vi "ClassAttributes_AddClassAttributes.vi"(7 "Action":T3=enum."GeneratePattern", 8 "error in (no error)":errorcluster, 10 "DataIn":variant, 11 "ClassRefToActOn":refnum<vi>) -> (0 "error out":errorcluster, 1 "Name":string, 2 "DataOut":variant, 3 "Cancelled":bool)   [LabVIEW 2020]
uses:
  Provider_BaseClassInterface/BaseProvider_SubVIs/BaseProvider_DesignPatternsActions.ctl
  Common/CommonVIs/CommonVIs_AttributeDataType.ctl
  Common/LvClass_class/GDSLvClass_ProviderTypes.ctl
  Provider_EndevoGOOP400/EndevoG4ProviderName.ctl
  Common/ScriptingFunctions/Scripting_ConnectorPanePatternType.ctl
  <vilib>/picture/picture.llb/imagedata.ctl
  Provider_LvNativeClass/ClassWriterNative_class/ClassWriterNative.lvclass
  Provider_BaseClassInterface/CreateMethodData.ctl
  Provider_EndevoGOOP300/GOOP300_SubVIs/GOOP300_MethodScopeType.ctl
  Provider_LvNativeClass/ClassWriterNative_class/IconDetails.ctl
  Provider_LvNativeClass/ClassWriterNative_class/IconSize.ctl
  Provider_BaseClassInterface/ClassWriter_class/ClassWriter.lvclass
panel:
  in  "_Cancel":bool
  in  "_OK":bool
  in  "ProcessName":T2(array[cluster]) caption="Attributes to add (can be empty)\nName                                        Array?      Data Type" {"Array?" items=["No", "1D", "2D", "3D"]}
  # "Class Attributes"
  # "Create"
  # "Get"
  # "Set"
  # "method"
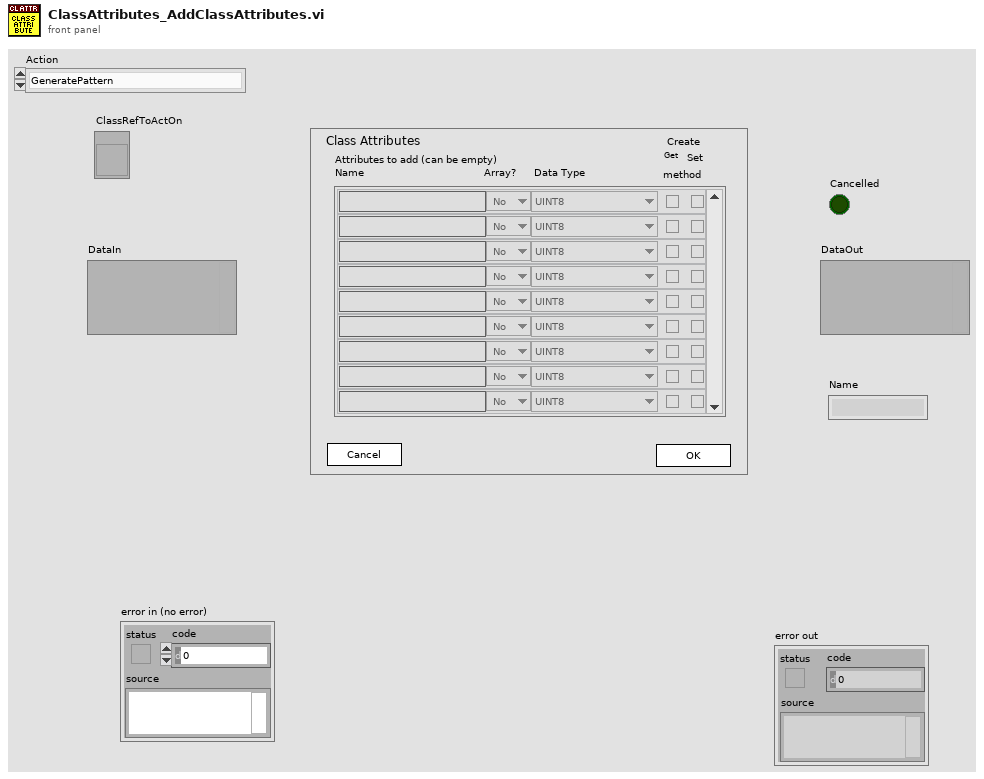
[diagram p1: front panel]
types:
  T1 = typedef "CommonVIs_AttributeDataType.ctl" = enum16{"UINT8", "INT8", "UINT16", "INT16", "UINT32", "INT32", "UINT64", "INT64", "SGL", "DBL", "EXT", "CSG", "CDB", "CXT", "TimeStamp", "STRING", "PATH", "BOOL", "ENUM", "RefNum", "VIRefNum", "LabVIEW Class", "Cluster", "Variant", "TypeDef", "Waveform", "LabVIEW Object", "Other", "void", "Set", "Map"}
  T2 = cluster{"Name":string, "Array?":u16, "AttributeDataType":T1, "GetMethod":bool, "SetMethod":bool}[]
  T3 = typedef "BaseProvider_DesignPatternsActions.ctl" = enum16{"AddPatternDialog", "GeneratePattern", "RemovePattern", "CreatePatternMethod", "UpdatePattern"}
  T4 = typedef "GDSLvClass_ProviderTypes.ctl" = enum16{"UnKnown(LabVOOP)", "Native", "EndevoGOOP3", "OpenG(RootObject)", "OpenG(OpenG_Object)", "EndevoGOOP4", "JKI1"}
  T5 = cluster{"Application":refnum<vi>, "SupportFolder":path, "TemplateName":string, "ClassProvider":T4, "ProtectedFolder":path, "UtilsFolder":path, "ProtectedFolderRef":refnum<vi>, "UtilsFolderRef":refnum<vi>, "ClassName":string, "GetClassAttributes.vi":path, "ClassAttributes.ctl":path, "GetClassAttributesRef":refnum<vi>, "ClassAttributesRef":refnum<vi>, "ProcessIdRef":refnum<vi>, "Data":cluster{"Name":string, "Array?":u16, "AttributeDataType":T1, "GetMethod":bool, "SetMethod":bool}[], "Singleton":bool, "VI_ToFind":path, "MethodTemplate":path, "VI":refnum<vi>, "GetObjectStatus":path, "ClassAttrib":refnum<vi>}
  T6 = cluster{"ProcessName":cluster{"Name":string, "Array?":u16, "AttributeDataType":T1, "GetMethod":bool, "SetMethod":bool}[]}
  T7 = cluster{"Cancelled":bool, "Files":path[], "ClassPath":path, "DataOut":variant}
  T8 = typedef "EndevoG4ProviderName.ctl" = enum16{"EndevoGOOP400"}
  T9 = enum32{"invalid lock state", "Not Locked", "Locked (No Password)", "Password-protected"}
  T10 = typedef "imagedata.ctl" = cluster{"image type":i32, "image depth":i32, "image":u8[], "mask":u8[], "colors":u32[], "Rectangle":cluster{"left":i16, "top":i16, "right":i16, "bottom":i16}}
  T11 = cluster{"AttributeNames":string[], "PropertyNode":bool, "FolderNames":string[]}
  T12 = typedef "ClassWriter.lvclass/CreateMethodData.ctl" = cluster{"MethodName":string, "RelativeMethodPath":path, "MethodDescription":string, "Scope/Visibility":T13, "MethodTemplateName":string, "IconOut":u8[][], "RelativeProjectClassPath":string, "OpenViAfterCreation":bool, "DynamicDispatchVi":bool, "ExtraCreateParameters":variant, "MustOverride":bool, "MustCallParent":bool, "IconDetails":T14, "AF-Option":variant, "TemplatePath":path}
  T13 = typedef "GOOP300_MethodScopeType.ctl" = enum16{"Use Parent Folder Scope", "Public", "Protected", "Private", "Community"}
  T14 = typedef "ClassWriterNative.lvclass/IconDetails.ctl" = cluster{"IconSize":T15, "ImageRows(32)":i32, "ConnectorPaneHeight":i32[]}
  T15 = typedef "ClassWriterNative.lvclass/IconSize.ctl" = enum16{"Full", "1 c-term high", "2 c-term high", "3 c-term high"}
  T16 = typedef "GDSLvCLass_ClassSettingsType.ctl" = cluster{"ClassProviderName":string, "ClassTemplateUsed":string, "ClassTemplateVersion":string, "ClassDescription":string, "PlugIns":T17[], "ConnectorPanePattern":string}
  T17 = typedef "GDSLvClass_PlugIn.ctl" = cluster{"Type":T18, "ID":string, "Version":string, "Path":path, "Name":string, "Data":variant}
  T18 = typedef "GDSLvClass_PlugInTypes.ctl" = enum16{"DesignPattern", "MethodTypes"}
  T19 = enum32{"invalid scope", "public", "private", "protected"}[]
  T20 = typedef "GOOP400_Options.ctl" = cluster{"FlatFolderStructure":bool}
  T21 = typedef "Scripting_ConnectorPanePatternType.ctl" = u16
  T22 = typedef "GDSLvClass_IconSettingsType.ctl" = cluster{"Frame":u32, "Frame thickness":u8, "Header Background":u32, "Header Text":u32, "ColorPublic":u32, "ColorProtected":u32, "ColorPrivate":u32, "Body Text":u32, "ClassBodyIcon":string}
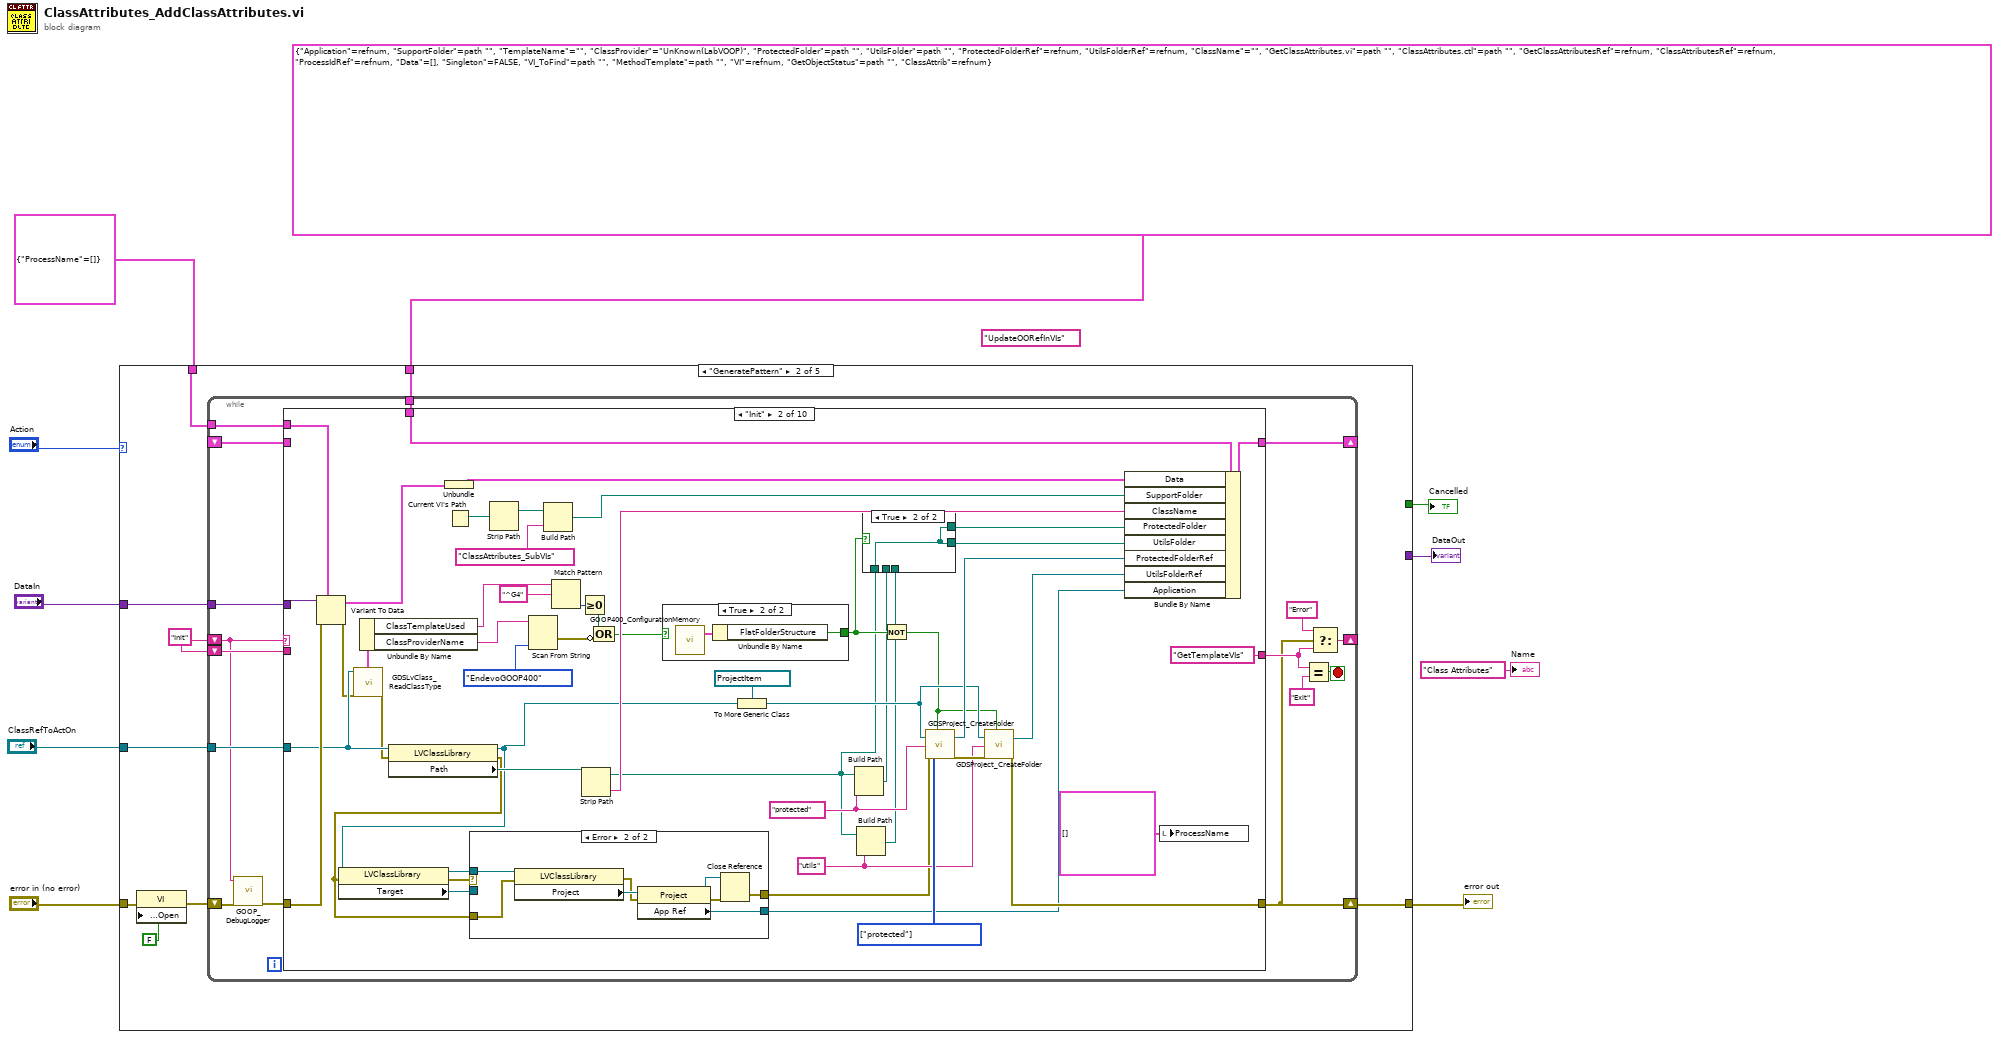
[diagram p0: block diagram]
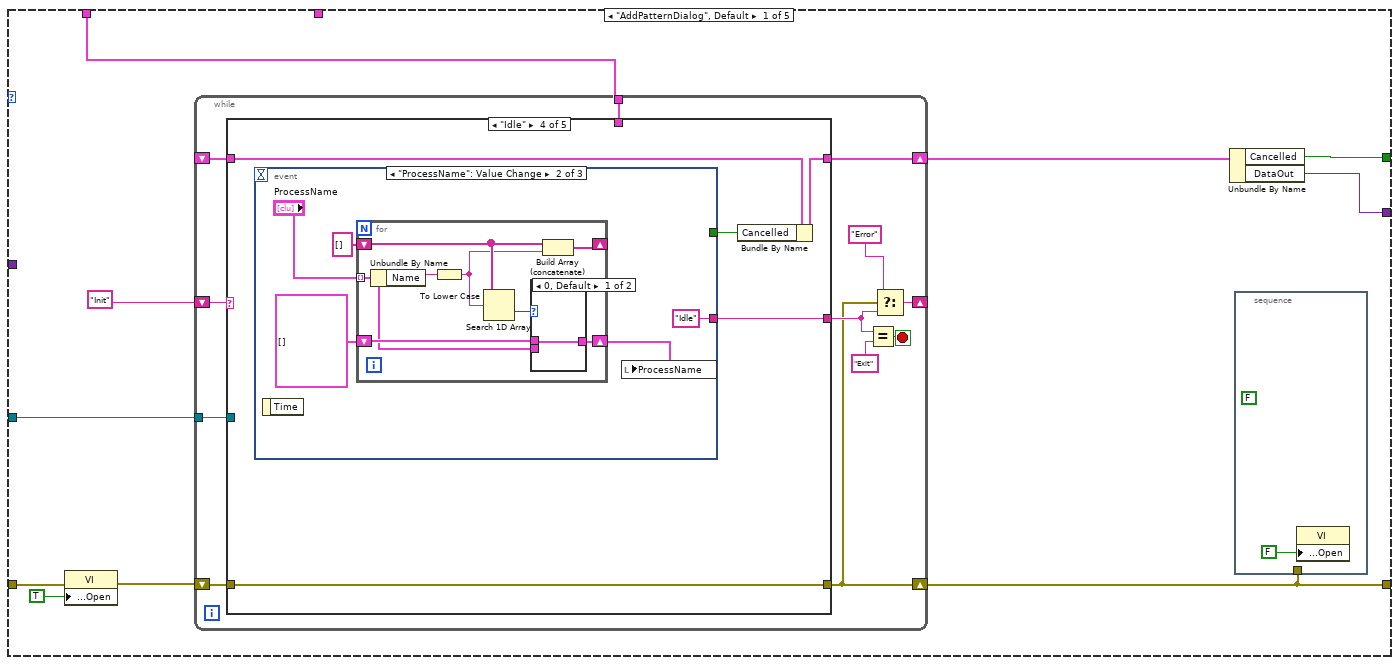
[diagram p2: hidden frame]
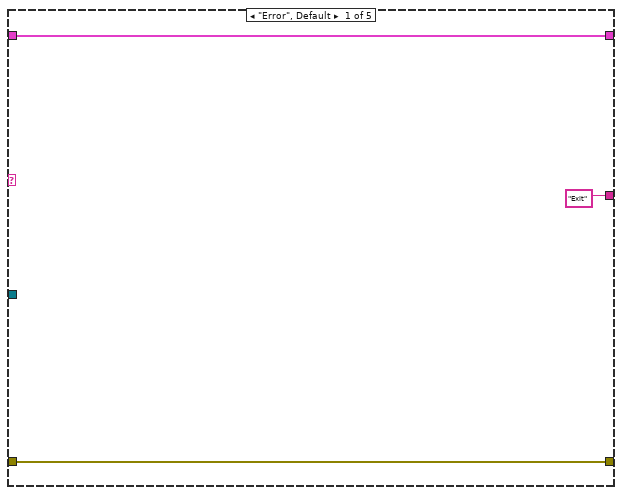
[diagram p3: hidden frame]
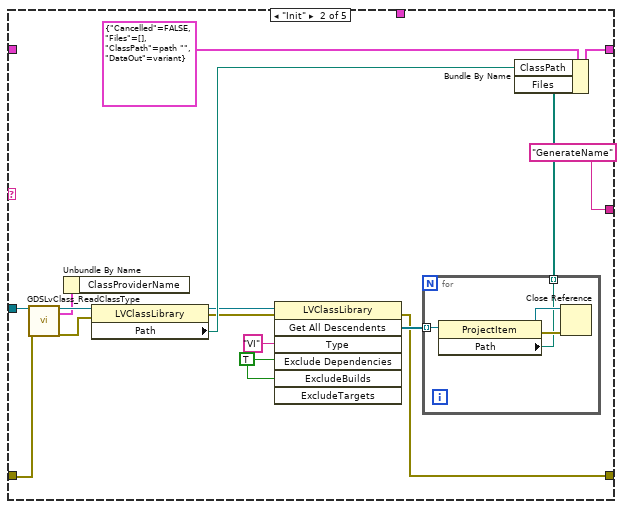
[diagram p4: hidden frame]
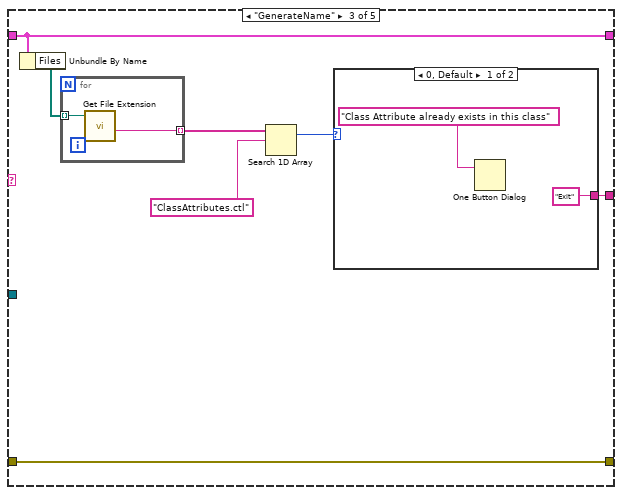
[diagram p5: hidden frame]
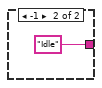
[diagram p6: hidden frame]
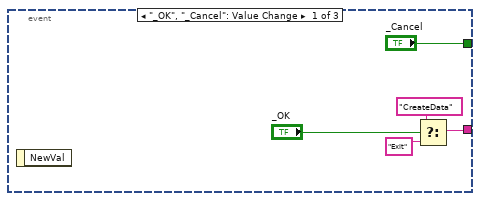
[diagram p7: hidden frame]
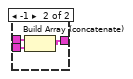
[diagram p8: hidden frame]
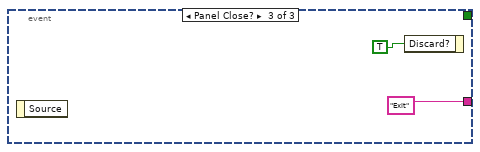
[diagram p9: hidden frame]
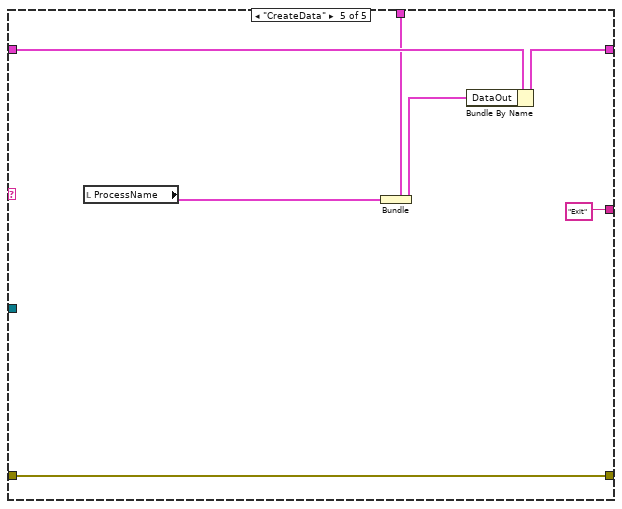
[diagram p10: hidden frame]
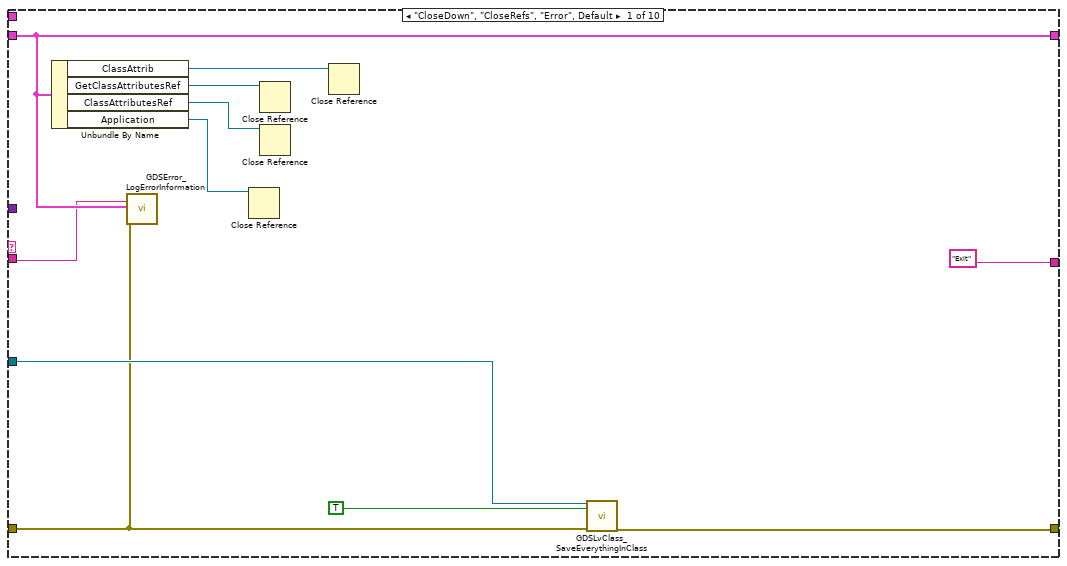
[diagram p11: hidden frame]
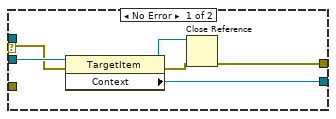
[diagram p14: hidden frame]
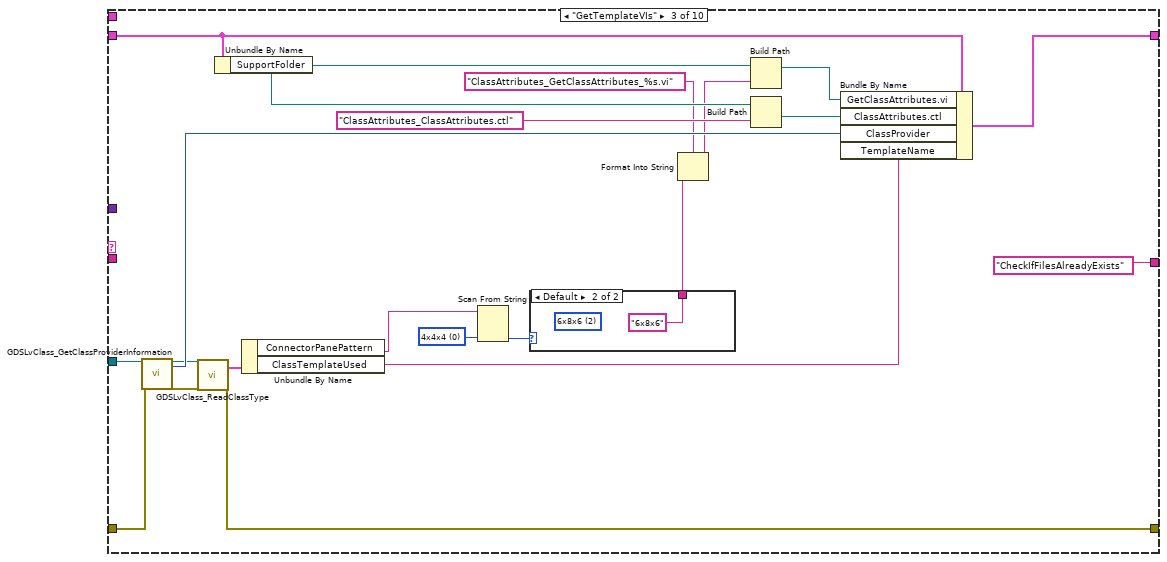
[diagram p15: hidden frame]
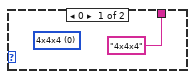
[diagram p16: hidden frame]
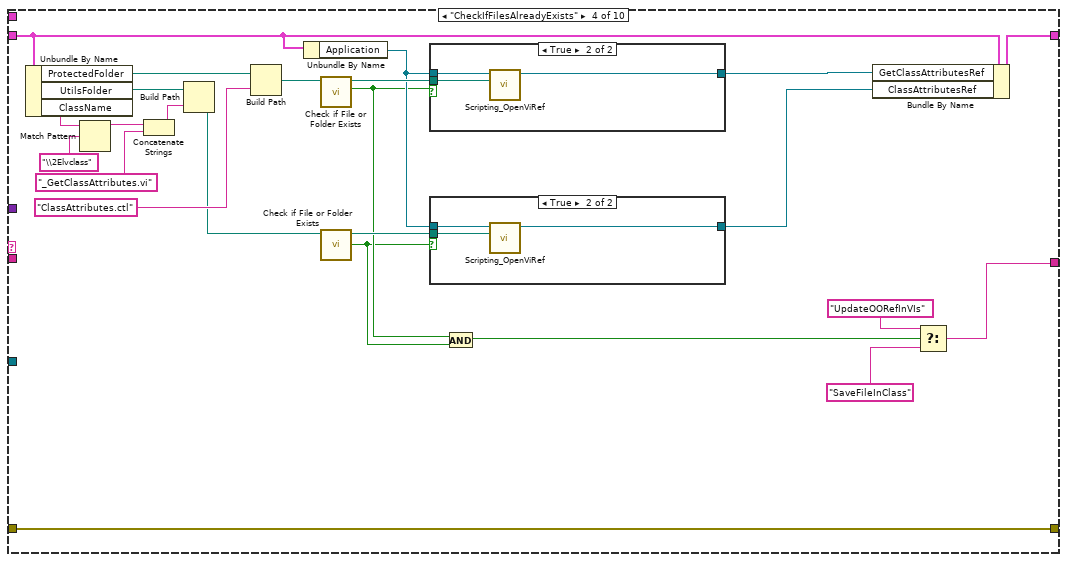
[diagram p17: hidden frame]
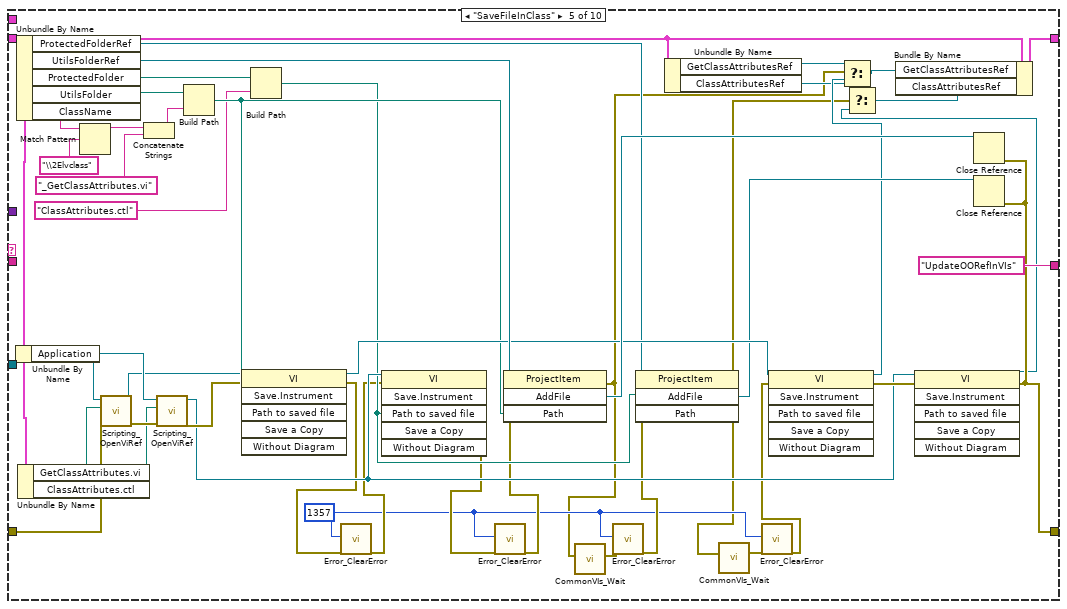
[diagram p20: hidden frame]
diagram:
  (unwired) "UpdateOORefInVIs"
  n1 = case shown="\"GeneratePattern\"" "Action" {
    tunnel: "error in (no error)" -> [w19 w107 w556 w647 w648]
    tunnel: [w16 w113 w562 w647 w648] -> w8
    tunnel: "ClassRefToActOn" -> [w14 w109 w558 _ _]
    tunnel: [w13 _ _ _ _] -> w6
    tunnel: [w12 _ _ _ _] -> w5
    tunnel: T6 {"ProcessName"=[]} ("output cluster") -> [w11 w111 w560 _ _]
    tunnel: "DataIn" -> [_ w112 w561 _ _]
    tunnel: T5 {"Application"=refnum, "SupportFolder"=path "", "TemplateName"="", "ClassProvider"=enum."UnKnown(LabVOOP)", "ProtectedFolder"=path "", "UtilsFolder"=path "", "ProtectedFolderRef"=refnum, "UtilsFolderRef"=refnum, "ClassName"="", "GetClassAttributes.vi"=path "", "ClassAttributes.ctl"=path "", "GetClassAttributesRef"=refnum, "ClassAttributesRef"=refnum, "ProcessIdRef"=refnum, "Data"=[], "Singleton"=FALSE, "VI_ToFind"=path "", "MethodTemplate"=path "", "VI"=refnum, "GetObjectStatus"=path "", "ClassAttrib"=refnum} -> [_ w110 w559 _ _]
    frame "AddPatternDialog", Default {
      n2 = property class="VI"(error in=w19, "Front Panel.Open"=TRUE ("Front Panel Window:Open")) -> (error out=w18:errorcluster)  [unwired: 1 in, 1 out]
      n3 = while {
        shift-right: [w26] -> w16
        shift-left: w18 -> [w33]
        shift-right: [w31] -> _
        shift-left: "Init" -> [w32]
        shift-right: [w25] -> w15
        shift-left: _ -> [w24]
        tunnel: w14 -> [w23]
        tunnel: w11 -> [w22]
        stop <- w30 stop-if-true
        n4 = case shown="\"Idle\"" w32 {
          tunnel: w33 -> [w36 w39 w60 w72 w100]
          tunnel: [w36 w48 w60 w72 w100] -> w26
          tunnel: ["Exit" "GenerateName" w62 w73 "Exit"] -> w27
          tunnel: [w34 w46 w61 w71 w102] -> w25
          tunnel: w24 -> [w34 _ w61 w69 w104]
          tunnel: w23 -> [_ w41 _ _ _]
          tunnel: w22 -> [_ _ _ _ w99]
          frame "Error", Default {
          }
          frame "Init" {
            w50 = TRUE ("ExcludeDependencies")
            n5 = call "GDSLvClass_ReadClassType.vi"("Class Refnum In"=w41, "error in (no error)"=w39) -> ("Class Refnum Out"=w40:refnum<vi>, "ClassSettings"=w37:T16, "error out"=w38:errorcluster)  [unwired: 15 in]
            n6 = Unbundle By Name(w37) -> ()  [unwired: 1 out]
            n7 = property class="LVClassLibrary"(reference=w40, error in=w38) -> (reference out=w43:refnum<vi>, error out=w42:errorcluster, "Path"=w45:path)
            n8 = invoke class="LVClassLibrary" method="Get All Descendents"(reference=w43, error in=w42, "Type"="VI", "Exclude Dependencies"=w50, "ExcludeBuilds"=w50) -> (error out=w48:errorcluster, "All Descendents"=w49:refnum<vi>[])  [unwired: 2 in, 5 out]
            n9 = for {
              tunnel: w49 -> [w56] mode=indexing
              tunnel: [w53] -> w44 mode=indexing
              n10 = property class="ProjectItem"(reference=w56) -> (reference out=w54:refnum<vi>, error out=w55:errorcluster, "Path"=w53:path)  [unwired: 1 in]
              n11 = Close Reference(reference=w54, error in (no error)=w55) -> ()  [unwired: 1 out]
            }
            n12 = Bundle By Name(cluster=T7 {"Cancelled"=FALSE, "Files"=[], "ClassPath"=path "", "DataOut"=variant}, "ClassPath"=w45, "Files"=w44) -> (w46:T7)
          }
          frame "GenerateName" {
            n13 = Unbundle By Name(w61) -> ("Files"=w63:path[])
            n14 = for {
              tunnel: w63 -> [w68] mode=indexing
              tunnel: [w67] -> w59 mode=indexing
              n15 = call <vilib>:"Get File Extension.vi"("file"=w68) -> ("filename without extension"=w67:string)  [unwired: 6 in, 4 out]
            }
            n16 = Search 1D Array(1D array=w59, element="ClassAttributes.ctl") -> (index of element=w57:i32)  [unwired: 1 in]
            n17 = case shown="0, Default" w57 {
              tunnel: ["Exit" "Idle"] -> w62
              frame 0, Default {
                n18 = One Button Dialog(message="Class Attribute already exists in this class") -> ()  [unwired: 1 in, 1 out]
              }
              frame -1 {
              }
            }
          }
          frame "Idle" {
            n19 = event shown="[1] \"ProcessName\": Value Change" {
              selector: _ -> [_ _ _]
              dyn-events: _ -> [_ _ _]
              timeout: _ -> [_ _ _]
              tunnel: [w77 "Idle" "Exit"] -> w73
              tunnel: ["_Cancel" _ _] -> w70
              event "_OK", "_Cancel": Value Change {
                n20 = event-data() -> ()  [unwired: 1 in, 1 out]
                n21 = Select(t="CreateData", s="_OK", f="Exit") -> (s? t:f=w77:string)
              }
              event "ProcessName": Value Change {
                n22 = event-data() -> ()  [unwired: 1 in, 1 out]
                n23 = for {
                  tunnel: "ProcessName" -> [w85] mode=indexing
                  shift-right: [w91] -> _
                  shift-left: string[] [] -> [w89]
                  shift-right: [w84] -> w79
                  shift-left: T2 [] -> [w86]
                  n24 = Unbundle By Name(w85) -> ("Name"=w90:string)
                  n25 = To Lower Case(string=w90) -> (all lower case string=w88:string)
                  n26 = Search 1D Array(1D array=w89, element=w88) -> (index of element=w87:i32)  [unwired: 1 in]
                  n27 = case shown="0, Default" w87 {
                    tunnel: w86 -> [w92 w95]
                    tunnel: w85 -> [_ w94]
                    tunnel: [w92 w93] -> w84
                    frame 0, Default {
                    }
                    frame -1 {
                      n28 = Build Array (concatenate)(w95, w94) -> (w93:T2)
                    }
                  }
                  n29 = Build Array (concatenate)(w89, w88) -> (w91:string[])
                }
                n30 = local write "ProcessName"(w79) -> ()
              }
              event Panel Close? {
                n31 = event-data() -> ()  [unwired: 1 in, 1 out]
                n32 = event-data("Discard?"=TRUE) -> ()  [unwired: 1 in, 1 out]
              }
            }
            n33 = Bundle By Name(cluster=w69, "Cancelled"=w70) -> (w71:T7)
          }
          frame "CreateData" {
            n34 = local read "ProcessName"() -> (w98:T2)
            n35 = Bundle(cluster=w99, "ProcessName"=w98) -> (w103:T6)
            n36 = Bundle By Name(cluster=w104, "DataOut"=w103) -> (w102:T7)
          }
        }
        n37 = Equal?(x=w27, y="Exit") -> (x = y?=w30:bool)
        n38 = Select(t="Error", s=w26, f=w27) -> (s? t:f=w31:string)
      }
      n39 = Unbundle By Name(w15) -> ("Cancelled"=w13:bool, "DataOut"=w12:variant)
      n40 = stacked-sequence {
        tunnel: w16 -> [_]
        frame #0 {
          (unwired) FALSE ("Visible")
          n41 = property class="VI"("Front Panel.Open"=FALSE ("Front Panel Window:Open")) -> ()  [unwired: 2 in, 2 out]
        }
      }
    }
    frame "GeneratePattern" {
      w105 = "Init"
      n42 = property class="VI"(error in=w107, "Front Panel.Open"=FALSE ("Front Panel Window:Open")) -> (error out=w106:errorcluster)  [unwired: 1 in, 1 out]
      n43 = while {
        shift-right: [w124] -> w113
        shift-left: w106 -> [w116]
        shift-right: [w129] -> _
        shift-left: w105 -> [w114]
        shift-right: [w123] -> _
        shift-left: _ -> [w122]
        tunnel: w112 -> [w121]
        tunnel: w111 -> [w120]
        tunnel: w110 -> [w119]
        tunnel: w109 -> [w118]
        shift-left: w105 -> [w117]
        stop <- w128 stop-if-true
        n44 = call "GOOP_DebugLogger.vi"("error in (no error)"=w116, "State"=w114) -> ("error out"=w115:errorcluster)  [unwired: 7 in, 2 out]
        n45 = case shown="\"Init\"" w114 {
          tunnel: w115 -> [w131 w185 w228 w247 w289 w318 w332 w357 w410 w501]
          tunnel: [w136 w174 w221 w247 w291 w312 w324 w356 w407 w486] -> w124
          tunnel: ["Exit" "GetTemplateVIs" "CheckIfFilesAlreadyExists" w233 "UpdateOORefInVIs" "UpdateAttributes" "UpdateIcons" "CreateMethods" w402 "CloseRefs"] -> w125
          tunnel: [w133 w189 w224 w243 w306 w319 w329 w359 w399 w485] -> w123
          tunnel: w122 -> [w133 _ w227 w244 w274 w319 w327 w359 w400 w485]
          tunnel: w121 -> [_ w188 _ _ _ _ _ _ _ _]
          tunnel: w120 -> [_ w187 _ _ _ _ _ _ _ _]
          tunnel: w119 -> [_ w186 _ _ _ _ _ _ _ _]
          tunnel: w118 -> [w135 w159 w229 _ _ w317 w336 w361 w406 w500]
          tunnel: w117 -> [w132 _ _ _ _ _ _ _ _ _]
          frame "CloseDown", "CloseRefs", "Error", Default {
            n46 = Unbundle By Name(w133) -> ("ClassAttrib"=w130:refnum<vi>, "GetClassAttributesRef"=w139:refnum<vi>, "ClassAttributesRef"=w138:refnum<vi>, "Application"=w134:refnum<vi>)
            n47 = call "GDSError_LogErrorInformation.vi"("State"=w132, "LocalVariableData"=w133, "error in (no error)"=w131) -> ()  [unwired: 16 in, 1 out]
            n48 = Close Reference(reference=w134) -> ()  [unwired: 1 in, 1 out]
            n49 = Close Reference(reference=w139) -> ()  [unwired: 1 in, 1 out]
            n50 = Close Reference(reference=w138) -> ()  [unwired: 1 in, 1 out]
            n51 = Close Reference(reference=w130) -> ()  [unwired: 1 in, 1 out]
            n52 = call "GDSLvClass_SaveEverythingInClass.vi"("ClassRefIn"=w135, "ForceResaving(False)"=TRUE, "error in"=w131) -> ("error out"=w136:errorcluster)  [unwired: 15 in, 1 out]
          }
          frame "Init" {
            w170 = "utils" ("name or relative path")
            w183 = T19 [enum."protected"] items=["invalid scope", "public", "private", "protected"] ("FolderScope")
            w182 = "protected" ("name or relative path")
            n53 = Variant To Data(error in=w185, type=w187, Variant=w188) -> (data=w169:T6, error out=w158:errorcluster)
            n54 = call "GDSLvClass_ReadClassType.vi"("Class Refnum In"=w159, "error in (no error)"=w158) -> ("ClassSettings"=w150:T16, "error out"=w157:errorcluster)  [unwired: 15 in, 1 out]
            n55 = Unbundle By Name(w150) -> ("ClassTemplateUsed"=w149:string, "ClassProviderName"=w148:string)
            n56 = property class="LVClassLibrary"(reference=w159, error in=w157) -> (reference out=w163:refnum<vi>, error out=w160:errorcluster, "Path"=w177:path)
            n57 = property class="LVClassLibrary"(reference=w163, error in=w160) -> (reference out=w166:refnum<vi>, error out=w164:errorcluster, "Target"=w165:refnum<vi>)
            n58 = Unbundle(w169) -> ("ProcessName"=w168:T2)
            n59 = Current VI's Path() -> (path=w181:path)
            n60 = case shown="Error" w164 {
              selector: w164 -> [w197 _]
              tunnel: w165 -> [w201 _]
              tunnel: [w200 w203] -> w162
              tunnel: [w196 w204] -> w161
              tunnel: w166 -> [_ w209]
              tunnel: w160 -> [_ w208]
              frame No Error {
                n61 = property class="TargetItem"(reference=w201, error in=w197) -> (reference out=w198:refnum<vi>, error out=w199:errorcluster, "Context"=w200:refnum<vi>)
                n62 = Close Reference(reference=w198, error in (no error)=w199) -> (error out=w196:errorcluster)
              }
              frame Error {
                n63 = property class="LVClassLibrary"(reference=w209, error in=w208) -> (error out=w202:errorcluster, "Project"=w207:refnum<vi>)  [unwired: 1 out]
                n64 = property class="Project"(reference=w207, error in=w202) -> (reference out=w205:refnum<vi>, error out=w206:errorcluster, "App Ref"=w203:refnum<vi>)
                n65 = Close Reference(reference=w205, error in (no error)=w206) -> (error out=w204:errorcluster)
              }
            }
            n66 = Strip Path(path=w181) -> (stripped path=w180:path)  [unwired: 1 out]
            n67 = Scan From String(input string=w148, default 1=EndevoG4ProviderName."EndevoGOOP400" ("ProviderName")) -> (error out=w154:errorcluster)  [unwired: 4 in, 2 out]
            n68 = Build Path(base path=w180, name or relative path="ClassAttributes_SubVIs") -> (appended path=w173:path)
            n69 = Match Pattern(string=w149, regular expression="^G4") -> (offset past match=w153:i32)  [unwired: 1 in, 3 out]
            n70 = Greater Or Equal To 0?(x=w153) -> (x >= 0?=w155:bool)
            n71 = Strip Path(path=w177) -> (stripped path=w142:path, name=w171:string)
            n72 = Compound Arithmetic op=OR(w155, invert w154) -> (w156:bool)
            n73 = case shown="True" w156 {
              tunnel: [_ w194] -> w147
              frame False {
              }
              frame True {
                n74 = call "GOOP400_ConfigurationMemory.vi"() -> ("OptionsOut"=w195:T20)  [unwired: 18 in, 1 out]
                n75 = Unbundle By Name(w195) -> ("FlatFolderStructure"=w194:bool)
              }
            }
            n76 = To More Generic Class(target class=refnum<vi> refnum ("AddItem"), reference=w163) -> (generic class reference=w175:refnum<vi>)
            n77 = Build Path(base path=w142, name or relative path=w182) -> (appended path=w146:path)
            n78 = Build Path(base path=w142, name or relative path=w170) -> (appended path=w145:path)
            n79 = case shown="True" w147 {
              tunnel: w146 -> [w191 _]
              tunnel: w145 -> [w192 _]
              tunnel: [w192 w193] -> w144
              tunnel: [w191 w193] -> w143
              tunnel: w142 -> [_ w193]
              frame False {
              }
              frame True {
              }
            }
            n80 = Not(x=w147) -> (.not. x?=w141:bool)
            n81 = call "GDSProject_CreateFolder.vi"("Project Item To Create Folder Below(Use MyComputer if not wired)"=w175, "FolderName"=w182, "error in (no error)"=w161, "FolderScope"=w183, "CreateThePhysicalFolderIfPossible(False)"=w141) -> ("ItemOut"=w178:refnum<vi>, "error out"=w176:errorcluster)  [unwired: 11 in, 2 out]
            n82 = call "GDSProject_CreateFolder.vi"("Project Item To Create Folder Below(Use MyComputer if not wired)"=w175, "FolderName"=w170, "error in (no error)"=w176, "CreateThePhysicalFolderIfPossible(False)"=w141) -> ("ItemOut"=w172:refnum<vi>, "error out"=w174:errorcluster)  [unwired: 12 in, 2 out]
            n83 = Bundle By Name(cluster=w186, "Data"=w168, "SupportFolder"=w173, "ClassName"=w171, "ProtectedFolder"=w143, "UtilsFolder"=w144, "ProtectedFolderRef"=w178, "UtilsFolderRef"=w172, "Application"=w162) -> (w189:T5)
            n84 = local write "ProcessName"(T2 [] ("ProcessName")) -> ()
          }
          frame "GetTemplateVIs" {
            w215 = T21 0 items=["4x4x4", "5x6x5", "6x8x6"] ("Pattern")
            n85 = call "GDSLvClass_GetClassProviderInformation.vi"("Class Refnum In"=w229, "error in (no error)"=w228) -> ("Class Refnum Out"=w223:refnum<vi>, "ClassProvider"=w225:T4, "error out"=w222:errorcluster)  [unwired: 15 in]
            n86 = call "GDSLvClass_ReadClassType.vi"("Class Refnum In"=w223, "error in (no error)"=w222) -> ("ClassSettings"=w220:T16, "error out"=w221:errorcluster)  [unwired: 15 in, 1 out]
            n87 = Unbundle By Name(w227) -> ("SupportFolder"=w218:path)
            n88 = Unbundle By Name(w220) -> ("ConnectorPanePattern"=w211:string, "ClassTemplateUsed"=w219:string)
            n89 = Scan From String(input string=w211, default 1=w215) -> (output 1=w212:T21)  [unwired: 3 in, 3 out]
            n90 = case shown="Default" w212 {
              tunnel: ["4x4x4" "6x8x6"] -> w210
              frame 0 {
                (unwired) T21 0 items=["4x4x4", "5x6x5", "6x8x6"] ("Pattern")
              }
              frame Default {
                (unwired) T21 2 items=["4x4x4", "5x6x5", "6x8x6"] ("Pattern")
              }
            }
            n91 = Format Into String(format string="ClassAttributes_GetClassAttributes_%s.vi" ("name or relative path"), w210) -> (resulting string=w213:string)  [unwired: 2 in, 1 out]
            n92 = Build Path(base path=w218, name or relative path=w213) -> (appended path=w226:path)
            n93 = Build Path(base path=w218, name or relative path="ClassAttributes_ClassAttributes.ctl") -> (appended path=w216:path)
            n94 = Bundle By Name(cluster=w227, "GetClassAttributes.vi"=w226, "ClassAttributes.ctl"=w216, "ClassProvider"=w225, "TemplateName"=w219) -> (w224:T5)
          }
          frame "CheckIfFilesAlreadyExists" {
            n95 = Unbundle By Name(w244) -> ("ProtectedFolder"=w250:path, "UtilsFolder"=w256:path, "ClassName"=w255:string)
            n96 = Match Pattern(string=w255, regular expression="\\2Elvclass") -> (before substring=w253:string)  [unwired: 1 in, 3 out]
            n97 = Concatenate Strings(w253, "_GetClassAttributes.vi" ("string")) -> (w251:string)
            n98 = Build Path(base path=w256, name or relative path=w251) -> (appended path=w246:path)
            n99 = Build Path(base path=w250, name or relative path="ClassAttributes.ctl") -> (appended path=w248:path)
            n100 = Unbundle By Name(w244) -> ("Application"=w240:refnum<vi>)
            n101 = call <vilib>:"Check if File or Folder Exists.vi"("path"=w248) -> ("file or folder exists?"=w238:bool, "dup path"=w245:path)  [unwired: 8 in, 1 out]
            n102 = call <vilib>:"Check if File or Folder Exists.vi"("path"=w246) -> ("file or folder exists?"=w237:bool, "dup path"=w241:path)  [unwired: 8 in, 1 out]
            n103 = case shown="True" w238 {
              tunnel: w240 -> [_ w262]
              tunnel: w245 -> [_ w261]
              tunnel: [_ w260] -> w242
              frame False {
              }
              frame True {
                n104 = call "Scripting_OpenViRef.vi"("ViPath/ViName/Viref"=w261, "AppRef"=w262) -> ("vi reference"=w260:refnum<vi>)  [unwired: 7 in, 2 out]
              }
            }
            n105 = case shown="True" w237 {
              tunnel: w240 -> [_ w259]
              tunnel: w241 -> [_ w258]
              tunnel: [_ w257] -> w239
              frame False {
              }
              frame True {
                n106 = call "Scripting_OpenViRef.vi"("ViPath/ViName/Viref"=w258, "AppRef"=w259) -> ("vi reference"=w257:refnum<vi>)  [unwired: 7 in, 2 out]
              }
            }
            n107 = And(x=w238, y=w237) -> (x .and. y?=w236:bool)
            n108 = Bundle By Name(cluster=w244, "GetClassAttributesRef"=w242, "ClassAttributesRef"=w239) -> (w243:T5)
            n109 = Select(t="UpdateOORefInVIs", s=w236, f="SaveFileInClass") -> (s? t:f=w233:string)
          }
          frame "SaveFileInClass" {
            w275 = 1357 ("code")
            n110 = Unbundle By Name(w274) -> ("Application"=w283:refnum<vi>)
            n111 = Unbundle By Name(w274) -> ("ProtectedFolderRef"=w293:refnum<vi>, "UtilsFolderRef"=w304:refnum<vi>, "ProtectedFolder"=w295:path, "UtilsFolder"=w307:path, "ClassName"=w302:string)
            n112 = Unbundle By Name(w274) -> ("GetClassAttributes.vi"=w288:path, "ClassAttributes.ctl"=w284:path)
            n113 = Match Pattern(string=w302, regular expression="\\2Elvclass") -> (before substring=w300:string)  [unwired: 1 in, 3 out]
            n114 = call "Scripting_OpenViRef.vi"("error in"=w289, "ViPath/ViName/Viref"=w288, "AppRef"=w283) -> ("error out"=w287:errorcluster, "vi reference"=w282:refnum<vi>)  [unwired: 6 in, 1 out]
            n115 = Concatenate Strings(w300, "_GetClassAttributes.vi" ("string")) -> (w298:string)
            n116 = call "Scripting_OpenViRef.vi"("error in"=w287, "ViPath/ViName/Viref"=w284, "AppRef"=w283) -> ("error out"=w286:errorcluster, "vi reference"=w285:refnum<vi>)  [unwired: 6 in, 1 out]
            n117 = Build Path(base path=w307, name or relative path=w298) -> (appended path=w296:path)
            n118 = invoke class="VI" method="Save.Instrument"(reference=w282, error in=w286, "Path to saved file"=w296) -> (reference out=w297:refnum<vi>, error out=w280:errorcluster)  [unwired: 3 in, 4 out]
            n119 = Build Path(base path=w295, name or relative path="ClassAttributes.ctl") -> (appended path=w281:path)
            n120 = call "Error_ClearError.vi"("code"=w275, "error in (no error)"=w280) -> ("error out"=w279:errorcluster)  [unwired: 16 in, 1 out]
            n121 = invoke class="VI" method="Save.Instrument"(reference=w285, error in=w279, "Path to saved file"=w281) -> (error out=w278:errorcluster)  [unwired: 3 in, 5 out]
            n122 = call "Error_ClearError.vi"("code"=w275, "error in (no error)"=w278) -> ("error out"=w277:errorcluster)  [unwired: 16 in, 1 out]
            n123 = invoke class="ProjectItem" method="AddFile"(reference=w304, error in=w277, "Path"=w296) -> (error out=w266:errorcluster, "AddFile"=w303:refnum<vi>)  [unwired: 1 in, 2 out]
            n124 = call "CommonVIs_Wait.vi"("error in"=w266) -> ("error out"=w265:errorcluster)  [unwired: 9 in]
            n125 = call "Error_ClearError.vi"("code"=w275, "error in (no error)"=w265) -> ("error out"=w276:errorcluster)  [unwired: 16 in, 1 out]
            n126 = invoke class="ProjectItem" method="AddFile"(reference=w293, error in=w276, "Path"=w281) -> (error out=w264:errorcluster, "AddFile"=w290:refnum<vi>)  [unwired: 1 in, 2 out]
            n127 = Unbundle By Name(w274) -> ("GetClassAttributesRef"=w272:refnum<vi>, "ClassAttributesRef"=w269:refnum<vi>)
            n128 = call "CommonVIs_Wait.vi"("error in"=w264) -> ("error out"=w263:errorcluster)  [unwired: 9 in]
            n129 = call "Error_ClearError.vi"("code"=w275, "error in (no error)"=w263) -> ("error out"=w267:errorcluster)  [unwired: 16 in, 1 out]
            n130 = invoke class="VI" method="Save.Instrument"(reference=w297, error in=w267) -> (reference out=w273:refnum<vi>, error out=w292:errorcluster)  [unwired: 4 in, 4 out]
            n131 = Select(t=w272, s=w266, f=w273) -> (s? t:f=w271:refnum<vi>)
            n132 = invoke class="VI" method="Save.Instrument"(reference=w285, error in=w292) -> (reference out=w270:refnum<vi>, error out=w291:errorcluster)  [unwired: 4 in, 4 out]
            n133 = Select(t=w269, s=w264, f=w270) -> (s? t:f=w268:refnum<vi>)
            n134 = Bundle By Name(cluster=w274, "GetClassAttributesRef"=w271, "ClassAttributesRef"=w268) -> (w306:T5)
            n135 = Close Reference(reference=w303, error in (no error)=w291) -> ()  [unwired: 1 out]
            n136 = Close Reference(reference=w290, error in (no error)=w291) -> ()  [unwired: 1 out]
          }
          frame "UpdateOORefInVIs" {
            n137 = property class="LVClassLibrary"(reference=w317) -> ("Path"=w315:path)  [unwired: 1 in, 2 out]
            n138 = Unbundle By Name(w319) -> ("GetClassAttributesRef"=w311:refnum<vi>)
            n139 = Build Array(w311) -> (w316:refnum<vi>[])
            n140 = Path To String(path=w315) -> (string=w314:string)
            n141 = for {
              tunnel: w316 -> [w320] mode=indexing
              shift-right: [w323] -> w312
              shift-left: w318 -> [w322]
              tunnel: w314 -> [w321]
              n142 = call "Scripting_ReplaceOORef.vi"("ViRef"=w320, "NewLvClassFile(ProjectPath or LvClassPath)"=w321, "error in (no error)"=w322) -> ("error out"=w323:errorcluster)  [unwired: 16 in]
            }
            n143 = invoke class="VI" method="Lock State.Set"(reference=w311, error in=w312, "lockState"=T9."Not Locked" ("Lock State")) -> (reference out=w309:refnum<vi>, error out=w308:errorcluster)  [unwired: 4 in, 5 out]
            n144 = invoke class="VI" method="User Edits.Allow"(reference=w309, error in=w308) -> ()  [unwired: 1 in, 3 out]
          }
          frame "UpdateAttributes" {
            n145 = Unbundle By Name(w327) -> ("Data"=w331:T2)
            n146 = Unbundle By Name(w327) -> ("GetClassAttributesRef"=w326:refnum<vi>)
            n147 = for {
              tunnel: w331 -> [w353] mode=indexing
              tunnel: [w352] -> w335 mode=indexing
              tunnel: [w351] -> w334 mode=indexing
              tunnel: [w350] -> w333 mode=indexing
              n148 = Unbundle By Name(w353) -> ("Name"=w352:string, "AttributeDataType"=w351:T1, "Array?"=w350:u16)  [unwired: 2 out]
            }
            n149 = Array Size(array=w331) -> (size(s)=w330:i32)
            n150 = case shown="1.." w330 {
              tunnel: w336 -> [_ w347]
              tunnel: w335 -> [_ w346]
              tunnel: w334 -> [_ w345]
              tunnel: w333 -> [_ w344]
              tunnel: w332 -> [w338 w342]
              tunnel: [w338 w341] -> w325
              tunnel: [_ w339] -> w328
              frame 0, Default {
              }
              frame 1.. {
                n151 = call "Scripting_PlaceControlsInClassAttribute.vi"("ClassRefnum"=w347, "ClassControl(if empty private member data will be used)"="ClassAttributes.ctl", "OpenVIWhileEditingAdnRetrunReference"=FALSE, "DeleteAllCurrentAttributesFirst(True)"=TRUE, "ControlNames"=w346, "DataTypes"=w345, "error in"=w342, "DeleteReferencesToCreatedAttributes(True)"=TRUE, "ArrayDimensions"=w344) -> ("Member Data"=w339:refnum<vi>, "error out"=w341:errorcluster)  [unwired: 4 in, 1 out]
              }
            }
            n152 = Bundle By Name(cluster=w327, "ClassAttrib"=w328) -> (w329:T5)
            n153 = call "Scripting_SaveUpdateSubVIs.vi"("error in (no error)"=w325, "VI Refnum"=w326) -> ("error out"=w324:errorcluster)  [unwired: 9 in]
          }
          frame "UpdateIcons" {
            w378 = u8 32 ("x")
            n154 = Unbundle By Name(w359) -> ("ClassAttributesRef"=w360:refnum<vi>, "GetClassAttributesRef"=w354:refnum<vi>)
            n155 = property class="LVClassLibrary"(reference=w361, error in=w357) -> (reference out=w366:refnum<vi>, error out=w362:errorcluster, "Member Data"=w364:refnum<vi>)
            n156 = call "GDSLvIcon_AnalyseViIcon.vi"("ViRef/LvCLassRef/LvLibRef/ViPath/2D_Image"=w364, "error in (no error)"=w362) -> ("HeaderIcon"=w367:u8[][], "error out"=w363:errorcluster)  [unwired: 5 in, 11 out]
            n157 = Close Reference(reference=w364, error in (no error)=w363) -> (error out=w365:errorcluster)
            n158 = Build Array(w360, w354) -> (w355:refnum<vi>[])
            n159 = Array Size(array=w367) -> (size(s)=w373:i32[])
            n160 = call "GDSLvClass_ReadClassColors.vi"("Library Refnum"=w366, "error in (no error)"=w365) -> ("LvClassIconSettings"=w369:T22, "error out"=w358:errorcluster)  [unwired: 12 in, 4 out]
            n161 = Unbundle By Name(w369) -> ("Frame"=w372:u32, "Body Text"=w371:u32, "Frame thickness"=w368:u8)
            n162 = Unbundle By Name(w369) -> ("ColorProtected"=w370:u32)
            n163 = Index Array(array=w373) -> (element #1=w375:i32)  [unwired: 2 in, 1 out]
            n164 = Multiply(x=w368, y=u8 2) -> (x*y=w376:u8)
            n165 = Add(x=w375, y=w376) -> (x+y=w377:i32)
            n166 = Increment(x=w377) -> (x+1=w379:i32)
            n167 = Subtract(x=w378, y=w379) -> (x-y=w380:i32)
            n168 = Subtract(x=w378, y=w376) -> (x-y=w381:u8)
            n169 = for {
              tunnel: w381 -> [_]
              tunnel: w380 -> [_]
              tunnel: w372 -> [w396]
              tunnel: w371 -> [_]
              tunnel: w370 -> [_]
              tunnel: w368 -> [w395]
              tunnel: w367 -> [w394]
              shift-right: [w387] -> w356
              shift-left: w358 -> [w386]
              tunnel: w355 -> [w383] mode=indexing
              n170 = call "GDSLvIcon_AnalyseViIcon.vi"("ViRef/LvCLassRef/LvLibRef/ViPath/2D_Image"=w383, "error in (no error)"=w386) -> ("BodyIcon"=w384:u8[][], "error out"=w385:errorcluster)  [unwired: 5 in, 11 out]
              n171 = call "GDSLvIcon_CreateIconPicture.vi"("FrameColor"=w396, "FrameThickness(1)"=w395, "HeaderIconIn"=w394, "BodyIconIn"=w384, "error in (no error)"=w385) -> ("WholeIconOut"=w389:u8[][], "error out"=w392:errorcluster)  [unwired: 9 in, 4 out]
              n172 = Reshape Array(w389, 1024 ("dimension size")) -> (w391:u8[])
              n173 = Bundle By Name(cluster=T10 {"image type"=0, "image depth"=8, "image"=[], "mask"=[], "colors"=[], "Rectangle"={"left"=0, "top"=0, "right"=32, "bottom"=32}} ("image data"), "image"=w391) -> (w393:T10)
              n174 = invoke class="VI" method="VI Icon.Set from Image Data"(reference=w383, error in=w392, "ImageData"=w393) -> (error out=w387:errorcluster)  [unwired: 3 in, 5 out]
            }
          }
          frame "CreateMethods" {
            n175 = Unbundle By Name(w400) -> ("Data"=w427:T2)
            n176 = call "CreateWriterFromClass.vi"("ClassPath/LvClassRef"=w406, "error in"=w410) -> ("ClassWriter"=w420:refnum<class "ClassWriter.lvclass">, "LVClassRef"=w418:refnum<vi>, "error out"=w421:errorcluster)  [unwired: 15 out]
            n177 = for {
              tunnel: w427 -> [w437] mode=indexing
              shift-right: [w430] -> w426
              shift-left: string[] [] -> [w431]
              n178 = Unbundle By Name(w437) -> ("Name"=w432:string, "GetMethod"=w436:bool, "SetMethod"=w433:bool)
              n179 = case shown="True" w436 {
                tunnel: w432 -> [w444 _]
                tunnel: [w442 _] -> w435
                frame True {
                  n180 = Format Into String(format string="Get%s", w444) -> (resulting string=w443:string)  [unwired: 2 in, 1 out]
                  n181 = Build Array(w443) -> (w442:string[])
                }
                frame False {
                }
              }
              n182 = case shown="True" w433 {
                tunnel: w432 -> [w440 _]
                tunnel: [w438 _] -> w434
                frame True {
                  n183 = Format Into String(format string="Set%s", w440) -> (resulting string=w439:string)  [unwired: 2 in, 1 out]
                  n184 = Build Array(w439) -> (w438:string[])
                }
                frame False {
                }
              }
              n185 = Build Array (concatenate)(w431, w435, w434) -> (w430:string[])
            }
            n186 = call "GDSLvClass_ReadClassType.vi"("Class Refnum In"=w418, "error in (no error)"=w421) -> ("ClassSettings"=w415:T16)  [unwired: 17 out]
            n187 = Unbundle By Name(w415) -> ("ClassTemplateUsed"=w416:string)
            n188 = Empty String/Path?(string/path=w416) -> (empty?=w413:bool)
            n189 = To More Specific Class(target class=refnum<class "ClassWriterNative.lvclass"> refnum ("reference in"), reference=w420, error in=w421) -> (specific class reference=w423:refnum<class "ClassWriterNative.lvclass">)  [unwired: 1 out]
            n190 = Select(t="BaseTemplate", s=w413, f=w416) -> (s? t:f=w417:string)
            n191 = call-dynamic "GetTemplatePath.vi"("reference in"=w423, "ClassTemplateSubDirectory"=w417, "error in (no error)"=w421) -> ("reference out"=w411:refnum<class "ClassWriterNative.lvclass">, "MethodTemplatePathOut"=w419:path, "error out"=w424:errorcluster)  [unwired: 14 out]
            n192 = call "GetClassTemplateMethods.vi"("MethodTemplatePath"=w419, "error in"=w424) -> ("PropertyMethodPaths"=w409:path[], "error out"=w412:errorcluster)  [unwired: 16 out]
            n193 = for {
              tunnel: w406 -> [w470]
              shift-right: [w472] -> w429
              shift-left: w412 -> [w469]
              shift-right: [w471] -> w428
              shift-left: w411 -> [w468]
              tunnel: w426 -> [w459] mode=indexing
              tunnel: w409 -> [w463]
              n194 = Match Pattern(string=w459, regular expression="^[Ss][Ee][Tt]") -> (offset past match=w461:i32)  [unwired: 1 in, 3 out]
              n195 = String Subset(string=w459, offset (0)=3) -> (substring=w451:string)  [unwired: 1 in]
              n196 = Greater Or Equal To 0?(x=w461) -> (x >= 0?=w457:bool)
              n197 = Boolean To (0,1)(Boolean=w457) -> (0, 1=w460:i16)
              n198 = Index Array(array=w463, index=w460) -> (element=w465:path)
              n199 = Strip Path(path=w465) -> (name=w464:string)  [unwired: 1 out]
              n200 = Concatenate Strings("ClassAttribute§" ("format string"), w451) -> (w449:string)
              n201 = Select(t="This method reads the class attribute %s" ("format string"), s=w457, f="This method writes the class attribute %s" ("format string")) -> (s? t:f=w454:string)
              n202 = Build Array(w449) -> (w447:string[])
              n203 = Format Into String(format string=w454, w451) -> (resulting string=w453:string)  [unwired: 2 in, 1 out]
              n204 = Bundle(cluster=T11 {"AttributeNames"=[], "PropertyNode"=FALSE, "FolderNames"=[]}, "AttributeNames"=w447) -> (w448:T11)  [unwired: 2 in]
              n205 = Bundle By Name(cluster=T12 {"MethodName"="", "RelativeMethodPath"=path "", "MethodDescription"="", "Scope/Visibility"=enum."Public", "MethodTemplateName"="", "IconOut"=[], "RelativeProjectClassPath"="", "OpenViAfterCreation"=FALSE, "DynamicDispatchVi"=FALSE, "ExtraCreateParameters"=variant, "MustOverride"=FALSE, "MustCallParent"=FALSE, "IconDetails"={"IconSize"=enum."Full", "ImageRows(32)"=0, "ConnectorPaneHeight"=[]}, "AF-Option"=variant, "TemplatePath"=path ""} ("CreateMethodData"), "ExtraCreateParameters"=w448, "MethodName"=w459, "MethodDescription"=w453, "MethodTemplateName"=w464, "DynamicDispatchVi"=FALSE) -> (w466:T12)
              n206 = call-dynamic "CreateMethod.vi"("ClassWriterNative.lvclass"=w468, "ClassItemRefIn"=w470, "CreateMethodData"=w466, "error in (no error)"=w469) -> ("ClassWriterNative.lvclass 2"=w471:refnum<class "ClassWriterNative.lvclass">, "error out"=w472:errorcluster)  [unwired: 12 in, 2 out]
            }
            n207 = call-dynamic "Destroy.vi"("ClassWriterNative"=w428, "error in (no error)"=w429) -> ("error out"=w408:errorcluster)  [unwired: 17 in]
            n208 = call "GDSLvClass_GetClassMethod.vi"("Class Refnum In"=w406, "VINames"=string[] ["_GetObjectStatus.vi"], "error in (no error)"=w408) -> ("ViPaths"=w401:path[], "error out"=w407:errorcluster)  [unwired: 13 in, 2 out]
            n209 = Index Array(array=w401) -> (element=w398:path)  [unwired: 1 in]
            n210 = Bundle By Name(cluster=w400, "GetObjectStatus"=w398) -> (w399:T5)
            n211 = Empty String/Path?(string/path=w398) -> (empty?=w397:bool)
            n212 = Select(t="CloseRefs", s=w397, f="UpdateGetObjectStatus") -> (s? t:f=w402:string)
          }
          frame "UpdateGetObjectStatus" {
            n213 = Unbundle By Name(w485) -> ("Application"=w484:refnum<vi>)
            n214 = Unbundle By Name(w485) -> ("GetObjectStatus"=w482:path, "ProtectedFolder"=w518:path)
            n215 = call "GDSLvClass_GetClassMethod.vi"("Class Refnum In"=w500, "VINames"=string[] ["_GetClassAttributes.vi"] ("VIsToSerachFor/ViName"), "error in (no error)"=w501) -> ("ViPaths"=w502:path[], "error out"=w483:errorcluster)  [unwired: 13 in, 2 out]
            n216 = Index Array(array=w502) -> (element #1=w505:path, element #2=w504:path)  [unwired: 2 in]
            n217 = call "Scripting_OpenViRef.vi"("error in"=w483, "ViPath/ViName/Viref"=w482, "AppRef"=w484) -> ("error out"=w480:errorcluster, "vi reference"=w479:refnum<vi>)  [unwired: 6 in, 1 out]
            n218 = Empty String/Path?(string/path=w505) -> (empty?=w503:bool)
            n219 = invoke class="VI" method="Lock State.Set"(reference=w479, error in=w480, "lockState"=T9."Not Locked" ("Lock State")) -> (reference out=w478:refnum<vi>, error out=w477:errorcluster)  [unwired: 4 in, 5 out]
            n220 = Select(t=w504, s=w503, f=w505) -> (s? t:f=w493:path)
            n221 = call "Scripting_FindObjectsOnDiagram.vi"("ViRef(Ignored If Not Wired)"=w478, "NodeTypesToSearchFor"=string[] ["ClusterConstant"], "Don'tSearchSubStructures(False)"=TRUE, "error in (no error)"=w477) -> ("Nodes"=w475:refnum<vi>[], "error out"=w509:errorcluster)  [unwired: 14 in]
            n222 = for {
              tunnel: w475 -> [w552] mode=indexing
              shift-right: [w548] -> w476
              shift-left: w509 -> [w549]
              tunnel: [w547] -> w515 mode=indexing
              n223 = To More Specific Class(target class=refnum<vi> refnum ("WhileLoop"), reference=w552, error in=w549) -> (specific class reference=w551:refnum<vi>, error out=w550:errorcluster)
              n224 = property class="ClustCnst"(reference=w551, error in=w550) -> (error out=w548:errorcluster, "Label.Text"=w547:string)  [unwired: 1 out]
            }
            n225 = Empty String/Path?(string/path=w493) -> (empty?=w494:bool)
            n226 = Build Path(base path=w518, name or relative path="ClassAttributes.ctl") -> (appended path=w512:path)
            n227 = Search 1D Array(1D array=w515, element="ClassAttributes") -> (index of element=w516:i32)  [unwired: 1 in]
            n228 = Delete From Array(array=w475, index=w516) -> (deleted portion=w517:refnum<vi>, array with subset deleted=w474:refnum<vi>[])  [unwired: 1 in]
            n229 = invoke class="GObj" method="Replace"(reference=w517, error in=w476, "Path"=w512) -> (error out=w514:errorcluster, "Replace"=w513:refnum<vi>)  [unwired: 3 in, 4 out]
            n230 = Close Reference(reference=w513, error in (no error)=w514) -> (error out=w519:errorcluster)
            n231 = Close Reference(reference=w474, error in (no error)=w519) -> (error out=w495:errorcluster)
            n232 = call "Scripting_FindVisOnDiagram.vi"("ViRef"=w478, "VIsToSerachFor/ViName"=string[] ["_GetAttributes.vi$"], "error in (no error)"=w495) -> ("VisFound"=w497:refnum<vi>[], "error out"=w496:errorcluster)  [unwired: 15 in]
            n233 = for {
              tunnel: [w540] -> w498 mode=indexing
              shift-right: [w539] -> w473
              shift-left: w496 -> [w538]
              tunnel: w497 -> [w537] mode=indexing
              tunnel: w494 -> [w531]
              tunnel: w493 -> [w530]
              w535 = refnum<vi> refnum  # Node
              n234 = To More Specific Class(target class=w535, reference=w537) -> (specific class reference=w536:refnum<vi>)  [unwired: 1 in, 1 out]
              n235 = property class="Node"(reference=w536, error in=w538) -> ("Desc"=w534:string)  [unwired: 2 out]
              n236 = Equal?(x=w534, y="ClassAttribute") -> (x = y?=w532:bool)
              n237 = Compound Arithmetic op=AND(w532, invert w531) -> (w529:bool)
              n238 = case shown="True" w529 {
                tunnel: [_ w546] -> w540
                tunnel: [w541 w545] -> w539
                tunnel: w538 -> [w541 w544]
                tunnel: w537 -> [_ w543]
                tunnel: w530 -> [_ w542]
                frame False {
                }
                frame True {
                  n239 = invoke class="GObj" method="Replace"(reference=w543, error in=w544, "Path"=w542) -> (error out=w545:errorcluster, "Replace"=w546:refnum<vi>)  [unwired: 3 in, 4 out]
                }
              }
            }
            n240 = Close Reference(reference=w497, error in (no error)=w473) -> ()  [unwired: 1 out]
            n241 = Close Reference(reference=w498, error in (no error)=w473) -> ()  [unwired: 1 out]
            n242 = invoke class="VI" method="BD.Remove Bad Wires"(reference=w478, error in=w473) -> (reference out=w487:refnum<vi>, error out=w488:errorcluster)  [unwired: 1 in, 1 out]
            n243 = call "Scripting_FindNodeOnDiagram.vi"("ViRef(Ignored If Not Wired)"=w487, "NodeTypesToSearchFor"=string[] ["DisableStructure"], "error in (no error)"=w488) -> ("Nodes"=w492:refnum<vi>[], "error out"=w490:errorcluster)  [unwired: 15 in]
            n244 = for {
              tunnel: w492 -> [w528] mode=indexing
              shift-right: [w521] -> w491
              shift-left: w490 -> [w524]
              w526 = i16 0 ("number")
              w527 = refnum<vi> refnum  # DisableStructure
              n245 = To More Specific Class(target class=w527, reference=w528, error in=w524) -> (specific class reference=w522:refnum<vi>, error out=w523:errorcluster)
              n246 = To Word Integer(number=w526) -> (16bit integer=w525:i16)
              n247 = property class="DisableStructure"(reference=w522, error in=w523, "VisFrame"=w526, "ActiveFrame"=w525) -> (error out=w521:errorcluster)  [unwired: 1 out]
            }
            n248 = Close Reference(reference=w492, error in (no error)=w491) -> (error out=w486:errorcluster)
          }
        }
        n249 = Equal?(x=w125, y="Exit") -> (x = y?=w128:bool)
        n250 = Select(t="Error", s=w124, f=w125) -> (s? t:f=w129:string)
      }
    }
    frame "CreatePatternMethod" {
      w554 = "Init"
      n251 = property class="VI"(error in=w556, "Front Panel.Open"=FALSE ("Front Panel Window:Open")) -> (error out=w555:errorcluster)  [unwired: 1 in, 1 out]
      n252 = while {
        shift-right: [w570] -> w562
        shift-left: w555 -> [w577]
        shift-right: [w575] -> _
        shift-left: w554 -> [w576]
        shift-right: [w569] -> _
        shift-left: _ -> [w568]
        tunnel: w561 -> [w567]
        tunnel: w560 -> [w566]
        tunnel: w559 -> [w565]
        tunnel: w558 -> [w564]
        shift-left: w554 -> [w563]
        stop <- w574 stop-if-true
        n253 = case shown="\"Find_GetInstanceVI\"" w576 {
          tunnel: w577 -> [w606 w614 w641]
          tunnel: [w598 w612 w642] -> w570
          tunnel: [w596 "ReplaceGetClassAttributes" "Exit"] -> w571
          tunnel: [w609 w617 w644] -> w569
          tunnel: w568 -> [_ w617 w644]
          tunnel: w567 -> [w608 _ _]
          tunnel: w566 -> [_ _ _]
          tunnel: w565 -> [w607 _ _]
          tunnel: w564 -> [w599 w615 w643]
          tunnel: w563 -> [_ _ _]
          frame "Init" {
            n254 = Variant To Data(error in=w606, type=cluster{path, "VI":refnum<vi>, "Name":string} {path "", "VI"=refnum, "Name"=""} ("cluster"), Variant=w608) -> (data=w587:cluster{path, "VI":refnum<vi>, "Name":string}, error out=w588:errorcluster)
            n255 = Unbundle(w587) -> (w585:path, "VI"=w586:refnum<vi>)  [unwired: 1 out]
            n256 = call "GDSLvClass_ReadClassType.vi"("Class Refnum In"=w599, "error in (no error)"=w588) -> ("ClassSettings"=w605:T16, "error out"=w598:errorcluster)  [unwired: 15 in, 1 out]
            n257 = Unbundle By Name(w605) -> ("ConnectorPanePattern"=w604:string, "ClassTemplateUsed"=w603:string)
            n258 = To Lower Case(string=w603) -> (all lower case string=w601:string)
            n259 = case shown="\"0\", Default" w604 {
              tunnel: ["4x4x4" "6x8x6"] -> w583
              frame "0", Default {
              }
              frame "1", "2" {
              }
            }
            n260 = Match Pattern(string=w601, regular expression="singleton" ("search string")) -> (offset past match=w602:i32)  [unwired: 1 in, 3 out]
            n261 = Greater Or Equal To 0?(x=w602) -> (x >= 0?=w597:bool)
            n262 = Current VI's Path() -> (path=w594:path)
            n263 = Strip Path(path=w594) -> (stripped path=w593:path)  [unwired: 1 out]
            n264 = Format Into String(format string="ClassAttributes_ReadClassAttributes_%s.vi" ("name or relative path"), w583) -> (resulting string=w590:string)  [unwired: 2 in, 1 out]
            n265 = Build Path(base path=w593, name or relative path="ClassAttributes_SubVIs") -> (appended path=w581:path)
            n266 = Format Into String(format string="ClassAttributes_GetClassAttributes_%s.vi" ("name or relative path"), w583) -> (resulting string=w584:string)  [unwired: 2 in, 1 out]
            n267 = Build Path(base path=w581, name or relative path=w590) -> (appended path=w589:path)
            n268 = Build Path(base path=w581, name or relative path=w584) -> (appended path=w580:path)
            n269 = Select(t="Find_GetInstanceVI", s=w597, f="ReplaceGetClassAttributes") -> (s? t:f=w596:string)
            n270 = Bundle By Name(cluster=w607, "MethodTemplate"=w585, "VI"=w586, "SupportFolder"=w581, "VI_ToFind"=w589, "GetClassAttributes.vi"=w580) -> (w609:T5)
          }
          frame "Find_GetInstanceVI" {
            n271 = Unbundle By Name(w617) -> ("VI_ToFind"=w620:path, "VI"=w613:refnum<vi>)
            n272 = Build Array(w620) -> (w619:path[])
            n273 = call "GDSLvClass_GetClassMethod.vi"("Class Refnum In"=w615, "VINames"=string[] ["_GetInstance.vi$"] ("VIsToSerachFor/ViName"), "error in (no error)"=w614) -> ("ViPaths"=w626:path[], "error out"=w621:errorcluster)  [unwired: 13 in, 2 out]
            n274 = call "Scripting_FindVisOnDiagram.vi"("ViRef"=w613, "VIsToSerachFor/ViName"=w619, "error in (no error)"=w621) -> ("VisFound"=w623:refnum<vi>[], "error out"=w622:errorcluster)  [unwired: 15 in]
            n275 = Index Array(array=w626) -> (element=w618:path)  [unwired: 1 in]
            n276 = Index Array(array=w623) -> (element=w624:refnum<vi>)  [unwired: 1 in]
            n277 = invoke class="GObj" method="Replace"(reference=w624, error in=w622, "Path"=w618) -> (error out=w616:errorcluster, "Replace"=w625:refnum<vi>)  [unwired: 3 in, 4 out]
            n278 = Close Reference(reference=w623, error in (no error)=w616) -> ()  [unwired: 1 out]
            n279 = Close Reference(reference=w625, error in (no error)=w616) -> (error out=w612:errorcluster)
          }
          frame "ReplaceGetClassAttributes", Default {
            n280 = Unbundle By Name(w644) -> ("GetClassAttributes.vi"=w634:path, "VI"=w629:refnum<vi>)
            n281 = Build Array(w634) -> (w633:path[])
            n282 = call "GDSLvClass_GetClassMethod.vi"("Class Refnum In"=w643, "VINames"=string[] ["GetClassAttributes.vi$"] ("VIsToSerachFor/ViName"), "error in (no error)"=w641) -> ("ViPaths"=w631:path[], "error out"=w632:errorcluster)  [unwired: 13 in, 2 out]
            n283 = Index Array(array=w631) -> (element=w630:path)  [unwired: 1 in]
            n284 = call "Scripting_FindVisOnDiagram.vi"("ViRef"=w629, "VIsToSerachFor/ViName"=w633, "error in (no error)"=w632) -> ("VisFound"=w637:refnum<vi>[], "error out"=w636:errorcluster)  [unwired: 15 in]
            n285 = Index Array(array=w637) -> (element=w639:refnum<vi>)  [unwired: 1 in]
            n286 = invoke class="GObj" method="Replace"(reference=w639, error in=w636, "Path"=w630) -> (error out=w640:errorcluster, "Replace"=w638:refnum<vi>)  [unwired: 3 in, 4 out]
            n287 = Close Reference(reference=w637, error in (no error)=w640) -> ()  [unwired: 1 out]
            n288 = Close Reference(reference=w638, error in (no error)=w640) -> (error out=w635:errorcluster)
            n289 = invoke class="VI" method="Save.Instrument"(reference=w629, error in=w635) -> (error out=w642:errorcluster)  [unwired: 4 in, 5 out]
          }
        }
        n290 = Equal?(x=w571, y="Exit") -> (x = y?=w574:bool)
        n291 = Select(t="Error", s=w570, f=w571) -> (s? t:f=w575:string)
      }
    }
    frame "UpdatePattern" {
    }
    frame "RemovePattern" {
    }
  }
  "error out" <- w8
  "DataOut" <- w5
  "Cancelled" <- w6
  "Name" <- "Class Attributes" ("Name")
